vi "VM - List of Variables.vi"(6 "error in":errorcluster, 7 "reverse? (F)":bool, 8 "sort":enum16{"don't sort", "name", "alias", "type"}(ring), 9 "VC Handle":T1=-1) -> (0 "error out":errorcluster, 2 "variables info":T2[](array[typedef]), 3 "dup VC Handle":T1=-1)   [LabVIEW 2021]
doc: "This VI returns information about variables in the given context. Refer to the VI help for more details.\n\n<b>VC Handle</b> specifies the handle of the variable context from which to return a list of variables. To obtain a list of global variables, pass -1 to this input.\n\n::: CalcExpress Toolkit :::\nCopyright (c) 2000-2026 Konstantin Shifershteyn. All rights reserved."
uses:
  cetypes.llb/VarMan Variable Info Cluster.ctl
  cetypes.llb/VarMan Variable Context Handle.ctl
  cetypes.llb/VarMan Error Code.ctl
  cersrc/celveng32.dll
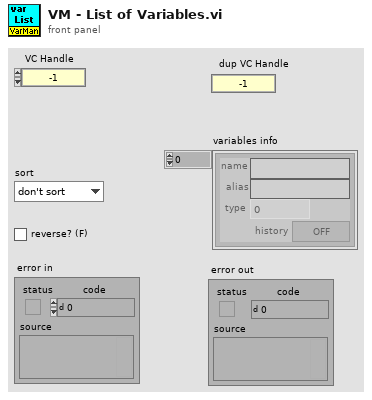
[diagram p1: front panel]
types:
  T1 = typedef "VarMan Variable Context Handle.ctl" = i32
  T2 = typedef "VarMan Variable Info Cluster.ctl" = cluster{"name":string, "alias":string, "type":u32, "history":bool}
  T3 = typedef "VarMan Error Code.ctl" = u16
  T4 = cluster{"name":string, "alias":string, "type":u32, "history":bool}[]
  T5 = cluster{"name":string, "alias":string, "type":u32, "history":bool}
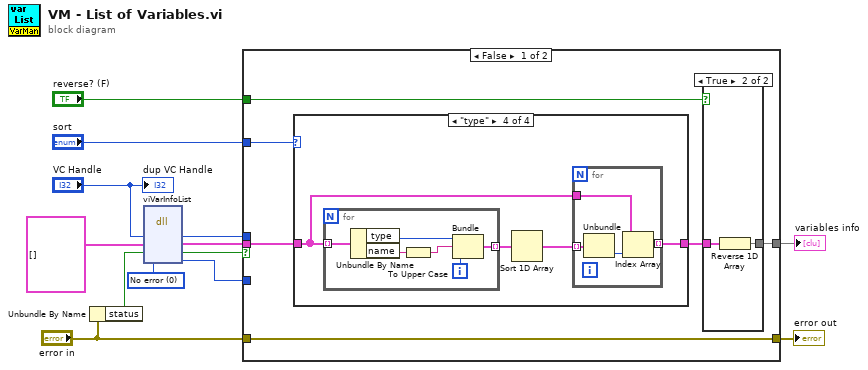
[diagram p0: block diagram]
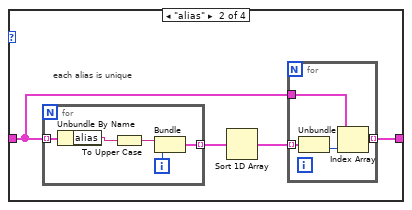
[diagram p3: hidden frame]
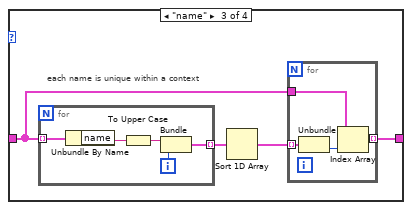
[diagram p4: hidden frame]
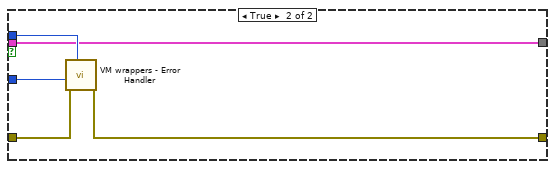
[diagram p6: hidden frame]
diagram:
  w3 = T3 0 items=["No error", "Invalid variable type", "Variable not found", "Variable already exists", "Invalid context handle", "Input error", "Invalid data format", "No history attached", "History already attached", "Invalid history parameters", "Wrong variable name", "Wrong alias name", "Non-unique alias", "Alias not found", "No alias associated", "Alias already associated", "Wrong context name", "Non-unique context name", "Context name not found", "Invalid parameter", "Generic error", "Memory Full", "Unrecognized LV error", "Unknown error code"] ("VarMan error")
  n1 = Unbundle By Name("error in") -> ("status"=w7:bool)
  n2 = dll-call lib="C:/LV Projects/CalcExpress 40 LV2021/vi.lib/addons/CalcExpress/cersrc/celveng*.dll" fn="viVarInfoList"("vch"="VC Handle", "vInfoList"=T4 [] ("variables info"), "errf"=w7, "errc"=w3) -> ("vch"=w9:T1, "vInfoList"=w4:T4, "errf"=w6:bool, "errc"=w5:T3)  [unwired: 4 in, 2 out]
  n3 = case shown="False" w6 {
    tunnel: [w19 w67] -> w13
    tunnel: w4 -> [w17 w67]
    tunnel: w5 -> [_ w64]
    tunnel: w9 -> [_ w68]
    tunnel: [w18 w65] -> w11
    tunnel: "error in" -> [w18 w66]
    tunnel: "sort" -> [w15 _]
    tunnel: "reverse? (F)" -> [w14 _]
    frame False {
      n4 = case shown="\"type\"" w15 {
        tunnel: [w20 w24 w37 w50] -> w16
        tunnel: w17 -> [w20 w21 w34 w47]
        frame "don't sort" {
        }
        frame "alias" {
          # "each alias is unique"
          n5 = for {
            tunnel: w21 -> [w33] mode=indexing
            tunnel: [w29] -> w22 mode=indexing
            i -> [w30]
            n6 = Unbundle By Name(w33) -> ("alias"=w32:string)
            n7 = To Upper Case(1:w32) -> (0:w31:string)
            n8 = Bundle(w31, w30) -> (w29:cluster{string, i32})  [unwired: 1 in]
          }
          n9 = Sort 1D Array(array=w22) -> (sorted array=w23:cluster{string, i32}[])
          n10 = for {
            tunnel: w23 -> [w28] mode=indexing
            tunnel: [w27] -> w24 mode=indexing
            tunnel: w21 -> [w25]
            n11 = Unbundle(w28) -> (w26:i32)  [unwired: 1 out]
            n12 = Index Array(array=w25, index=w26) -> (element=w27:T5)
          }
        }
        frame "name" {
          # "each name is unique within a context"
          n13 = for {
            tunnel: w34 -> [w46] mode=indexing
            tunnel: [w42] -> w35 mode=indexing
            i -> [w43]
            n14 = Unbundle By Name(w46) -> ("name"=w45:string)
            n15 = To Upper Case(1:w45) -> (0:w44:string)
            n16 = Bundle(w44, w43) -> (w42:cluster{string, i32})  [unwired: 1 in]
          }
          n17 = Sort 1D Array(array=w35) -> (sorted array=w36:cluster{string, i32}[])
          n18 = for {
            tunnel: w36 -> [w41] mode=indexing
            tunnel: [w40] -> w37 mode=indexing
            tunnel: w34 -> [w38]
            n19 = Unbundle(w41) -> (w39:i32)  [unwired: 1 out]
            n20 = Index Array(array=w38, index=w39) -> (element=w40:T5)
          }
        }
        frame "type" {
          n21 = for {
            tunnel: w47 -> [w60] mode=indexing
            tunnel: [w58] -> w48 mode=indexing
            i -> [w59]
            n22 = Unbundle By Name(w60) -> ("type"=w55:u32, "name"=w57:string)
            n23 = To Upper Case(1:w57) -> (0:w56:string)
            n24 = Bundle("type"=w55, w56, w59) -> (w58:cluster{"type":u32, string, i32})  [unwired: 1 in]
          }
          n25 = Sort 1D Array(array=w48) -> (sorted array=w49:cluster{"type":u32, string, i32}[])
          n26 = for {
            tunnel: w49 -> [w54] mode=indexing
            tunnel: [w53] -> w50 mode=indexing
            tunnel: w47 -> [w51]
            n27 = Unbundle(w54) -> (w52:i32)  [unwired: 2 out]
            n28 = Index Array(array=w51, index=w52) -> (element=w53:T5)
          }
        }
      }
      n29 = case shown="True" w14 {
        tunnel: w16 -> [w61 w63]
        tunnel: [w61 w62] -> w19
        frame False {
        }
        frame True {
          n30 = Reverse 1D Array(array=w63) -> (reversed array=w62:T4)
        }
      }
    }
    frame True {
      n31 = call "VM wrappers - Error Handler.vi"("VC Handle"=w68, "error before"=w66, "VarMan error"=w64) -> ("error out"=w65:errorcluster)  [unwired: 7 in, 1 out]
    }
  }
  "error out" <- w11
  "variables info" <- w13
  "dup VC Handle" <- "VC Handle"
